vi "VIH Utility - APP - Is Value Changed (DBL).vi"(6 "Changed at 1st call (T)":bool=TRUE, 7 "Value":dbl) -> (2 "Changed":bool, 3 "dup Value":dbl)   [LabVIEW 2014]
doc: "::: VI Helpeks :::\nCopyright (c) 2000-2026 Konstantin Shifershteyn. All rights reserved."
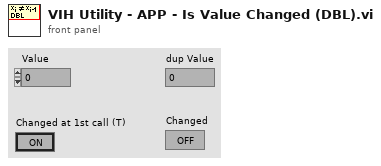
[diagram p1: front panel]
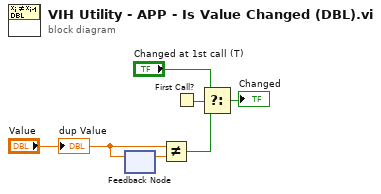
[diagram p0: block diagram]
diagram:
  n1 = feedback-in #1("Value") -> ()
  n2 = feedback #1() -> (w3:dbl)  [unwired: 1 in]
  n3 = Not Equal?(x="Value", y=w3) -> (x != y?=w1:bool)
  n4 = First Call?() -> (First Call?: T/F=w4:bool)
  n5 = Select(t="Changed at 1st call (T)", s=w4, f=w1) -> (s? t:f=→"Changed":bool)
  "dup Value" <- "Value"
